vi "pack frame.vi"(4 "switch bitrate? (F)":bool, 6 "can fd? (F)":bool, 7 "extended id?":bool, 8 "remote transmission request? (F)":bool, 10 "data":u8[](array[numeric]) format="%x", 11 "id":u32 format="%x") -> (3 "frame":u8[](array[numeric]) format="%x")   [LabVIEW 2024, in "atsj peakcan basic.lvlib"]
uses:
  atsj peakcan basic.lvlib
  message type.ctl
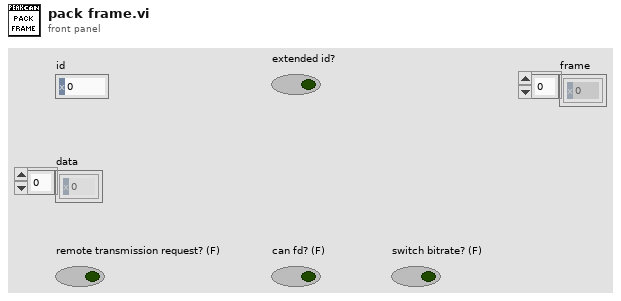
[diagram p1: front panel]
types:
  T1 = typedef "atsj peakcan basic.lvlib/message type.ctl" = cluster{"remote transmission request ":bool, "extended":bool, "fd":bool, "fd bit rate switch":bool, "fd error state":bool, "echo":bool, "error":bool, "status":bool}
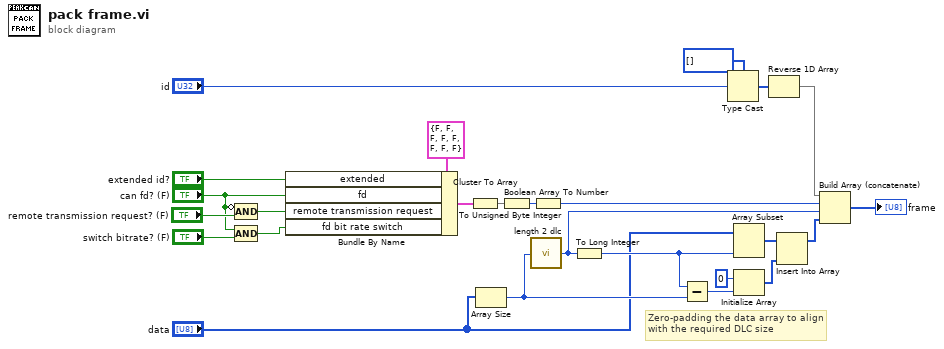
[diagram p0: block diagram]
diagram:
  # "Zero-padding the data array to align with the required DLC size"
  n1 = Compound Arithmetic op=AND(invert "can fd? (F)", "remote transmission request? (F)") -> (w4:bool)
  n2 = Compound Arithmetic op=AND("can fd? (F)", "switch bitrate? (F)") -> (w2:bool)
  n3 = Bundle By Name(cluster=T1 {"remote transmission request "=FALSE, "extended"=FALSE, "fd"=FALSE, "fd bit rate switch"=FALSE, "fd error state"=FALSE, "echo"=FALSE, "error"=FALSE, "status"=FALSE}, "extended"="extended id?", "fd"="can fd? (F)", "remote transmission request"=w4, "fd bit rate switch"=w2) -> (w10:T1)
  n4 = Cluster To Array(cluster=w10) -> (array=w13:bool[])
  n5 = Array Size(array="data") -> (size(s)=w7:i32)
  n6 = Boolean Array To Number(Boolean array=w13) -> (number=w14:u32)
  n7 = call "length 2 dlc.vi"("length"=w7) -> ("dlc"=w8:u8)
  n8 = To Unsigned Byte Integer(number=w14) -> (unsigned 8bit integer=w17:u8)
  n9 = To Long Integer(number=w8) -> (32bit integer=w23:i32)
  n10 = Subtract(x=w23, y=w7) -> (x-y=w20:i32)
  n11 = Type Cast(type=u8[] [], x="id") -> (*(type *) &x=w16:u8[])
  n12 = Array Subset(array="data", length=w23) -> (w21:u8[])  [unwired: 1 in]
  n13 = Initialize Array(u8 0, w20) -> (w22:u8[])
  n14 = Reverse 1D Array(array=w16) -> (reversed array=w18:u8[])
  n15 = Insert Into Array(array=w21, new element=w22) -> (w24:u8[])  [unwired: 1 in]
  n16 = Build Array (concatenate)(w18, w17, w8, w24) -> (→"frame":u8[])
